vi "Read Photodiode.vi"() -> (1 "Digital Vout":dbl, 2 "Analog  Vout":dbl)   [LabVIEW 2020]
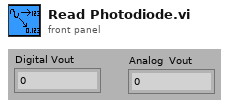
[diagram p1: front panel]
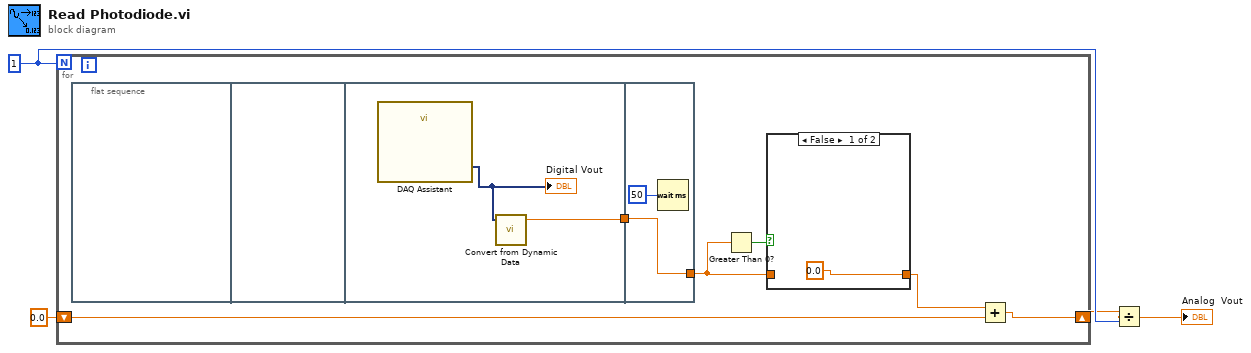
[diagram p0: block diagram]
diagram:
  w4 = 1
  n1 = for {
    N: w4 -> [_]
    shift-right: [w8] -> w2
    shift-left: 0.0 -> [w9]
    n2 = flat-sequence {
      tunnel: [w13] -> w10
      tunnel: [w15] -> w6
      tunnel: w10 -> [w15]
      frame #0 {
      }
      frame #1 {
      }
      frame #2 {
        n3 = call "DAQ Assistant"() -> ("data"=w14:dynamicdata)  [unwired: 17 in, 2 out]
        "Digital Vout" <- w14
        n4 = call "Convert from Dynamic Data"("Dynamic Data Type"=w14) -> ("Scalar"=w13:dbl)  [unwired: 3 in]
      }
      frame #3 {
        n5 = Wait (ms)(milliseconds to wait=u32 50) -> ()  [unwired: 1 out]
      }
    }
    n6 = Greater Than 0?(x=w6) -> (x > 0?=w7:bool)
    n7 = case shown="False" w7 {
      tunnel: [0.0 w12] -> w5
      tunnel: w6 -> [_ w12]
      frame False {
      }
      frame True {
      }
    }
    n8 = Add(x=w5, y=w9) -> (x+y=w8:dbl)
  }
  n9 = Divide(x=w2, y=w4) -> (x/y=→"Analog  Vout":dbl)
